vi "PicoScope2000aSetEtsTimeBuffer.vi"(8 "error in (no error)":errorcluster, 10 "bufferLth":i32, 11 "handle in":i16) -> (0 "error out":errorcluster, 2 "EtsTimeValues":i64[](array[numeric]), 3 "handle out":i16)   [LabVIEW 2009]
doc: "Calls SetEtsTimeBuffer"
uses:
  ps2000a.dll
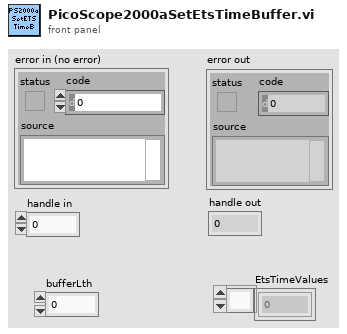
[diagram p1: front panel]
types:
  T1 = enum16{"U8", "I8", "U16", "I16", "U32", "I32", "U64", "I64"}
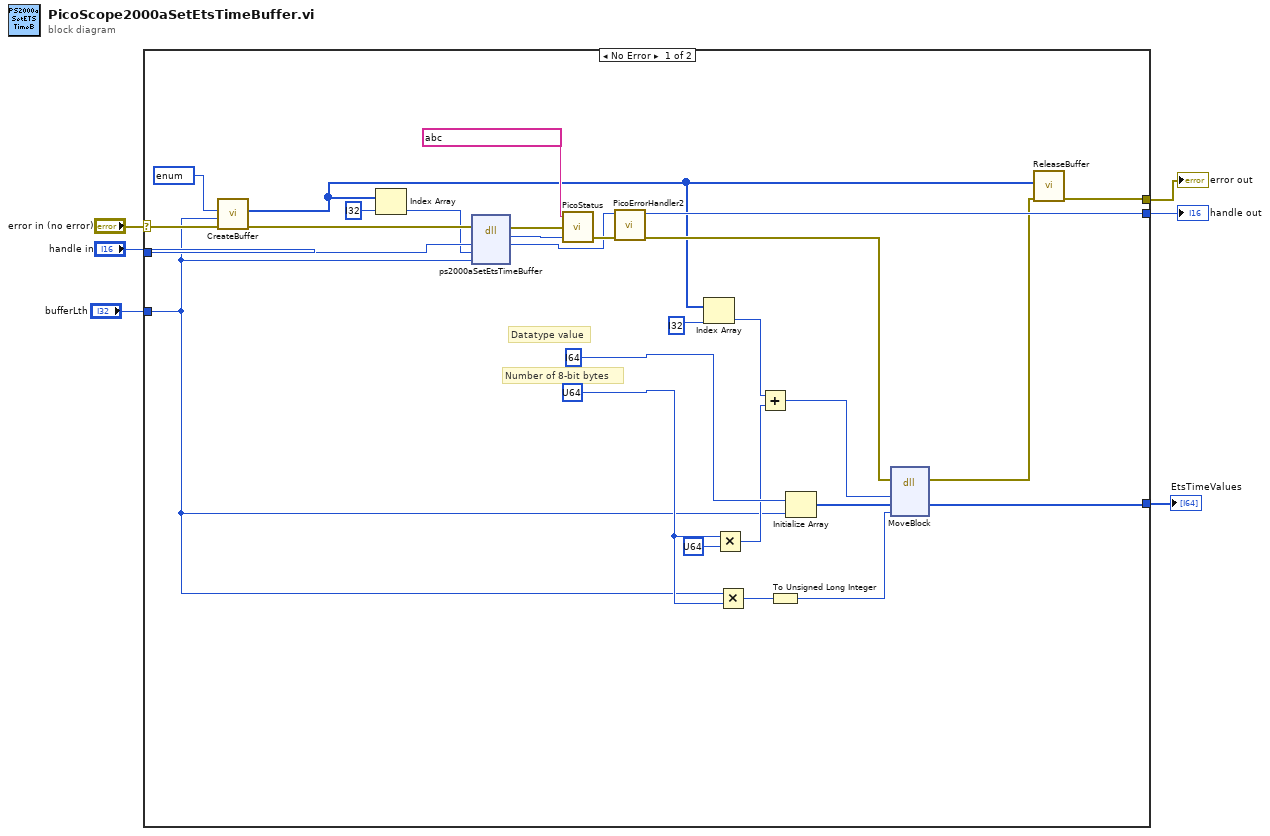
[diagram p0: block diagram]
diagram:
  n1 = case shown="No Error" "error in (no error)" {
    selector: "error in (no error)" -> [w27 w35]
    tunnel: [w25 w35] -> w4
    tunnel: "handle in" -> [w31 w34]
    tunnel: [w28 w34] -> w5
    tunnel: "bufferLth" -> [w9 _]
    tunnel: [w11 _] -> w1
    frame #0 {
      w19 = u64 ? ("y")
      # "Number of 8-bit bytes"
      # "Datatype value"
      n2 = call "CreateBuffer.vi"("error in (no error)"=w27, "Buffer size"=w9, "Data type"=T1 ?) -> ("error out"=w26:errorcluster, "Pointer and BufferSize"=w8:u64[])  [unwired: 7 in]
      n3 = Index Array(array=w8, index=i32 ?) -> (element=w24:u64)
      n4 = dll-call lib="ps2000a.dll" fn="ps2000aSetEtsTimeBuffer" ("ps3000.dll:_ps3000_open_unit@0")(error in=w26, "handle"=w31, "buffer"=w24, "bufferLth"=w9) -> (error out=w30:errorcluster, "PICO_STATUS"=w29:u32, "handle"=w28:i16)  [unwired: 4 in, 1 out]
      n5 = call "PicoStatus.vi"("PICO STATUS"=w29, "error in"=w30, "source"=string ?) -> ("error out"=w33:errorcluster)
      n6 = call "PicoErrorHandler2.vi"("error in (no error)"=w33, "handle In"=w28) -> ("error out"=w12:errorcluster)  [unwired: 9 in]
      n7 = Index Array(array=w8, index=i32 ?) -> (element=w21:u64)
      n8 = Multiply(x=w19, y=u64 ?) -> (x*y=w20:u64)
      n9 = Multiply(x=w9, y=w19) -> (x*y=w18:u64)
      n10 = Add(x=w21, y=w20) -> (x+y=w17:u64)
      n11 = To Unsigned Long Integer(number=w18) -> (unsigned 32bit integer=w15:u32)
      n12 = Initialize Array(i64 ? ("element"), w9) -> (w16:i64[])
      n13 = dll-call lib="LabVIEW" fn="MoveBlock"(error in=w12, "Source"=w17, "Destination"=w16, "Size"=w15) -> (error out=w13:errorcluster, "Destination"=w11:i64[])  [unwired: 5 in, 1 out]
      n14 = call "ReleaseBuffer.vi"("error in (no error)"=w13, "Pointer and BufferSize"=w8) -> ("error out"=w25:errorcluster)  [unwired: 9 in]
    }
    frame #1 {
    }
  }
  "error out" <- w4
  "handle out" <- w5
  "EtsTimeValues" <- w1
